vi "Utility - Set File List Icons.vi"(8 "error in":errorcluster, 11 "MCListbox Refnums":refnum<vi>[](array[refnum])) -> (0 "error out":errorcluster)   [LabVIEW 2014]
doc: "::: VI Helpeks :::\nCopyright (c) 2000-2026 Konstantin Shifershteyn. All rights reserved."
panel:
  # "VI Helpeks\nCopyright (c) 2012-2026 Konstantin Shifershteyn"
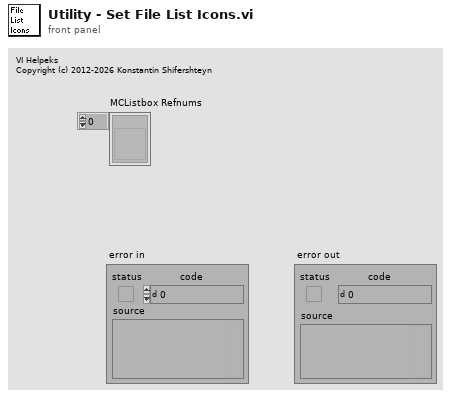
[diagram p1: front panel]
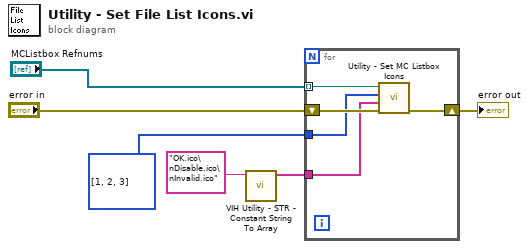
[diagram p0: block diagram]
diagram:
  n1 = call "VIH Utility - STR - Constant String To Array.vi"("String in"="OK.ico\nDisable.ico\nInvalid.ico") -> ("Array out"=w4:string[])  [unwired: 10 in]
  n2 = for {
    tunnel: w4 -> [w10]
    tunnel: i32[] [1, 2, 3] -> [w9]
    tunnel: "MCListbox Refnums" -> [w7] mode=indexing
    shift-right: [w8] -> w2
    shift-left: "error in" -> [w11]
    n3 = call "Utility - Set MC Listbox Icons.vi"("error in"=w11, "Icon Filenames"=w10, "Symbol Indices"=w9, "MCListbox Refnum"=w7) -> ("error out"=w8:errorcluster)  [unwired: 7 in]
  }
  "error out" <- w2
